vi "FT10xx系列_ITTR_sample_1.0.3.vi"() -> ()   [LabVIEW 2017]
uses:
  National Instruments/LabVIEW 2017/user.lib/smncsftmt/smncsftmt.lvlib
panel:
  in  "模式选择":enum32{"单选选项1", "单选选项2"}(radio)
  out "已连接？":bool
  in  "路径":path=path "D:/Siminics"
  out "error out":errorcluster caption="错误输出"
  in  "统计周期（us）":i32=1000
  in  "采集时间（s）":sgl=1.0
  # "FT10XX系列ITTR"
  # "时间停止："
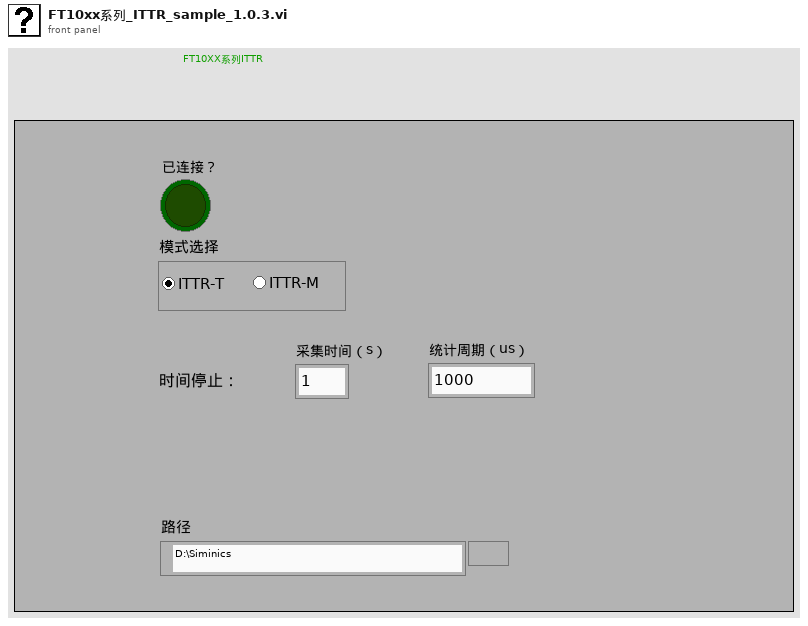
[diagram p1: front panel]
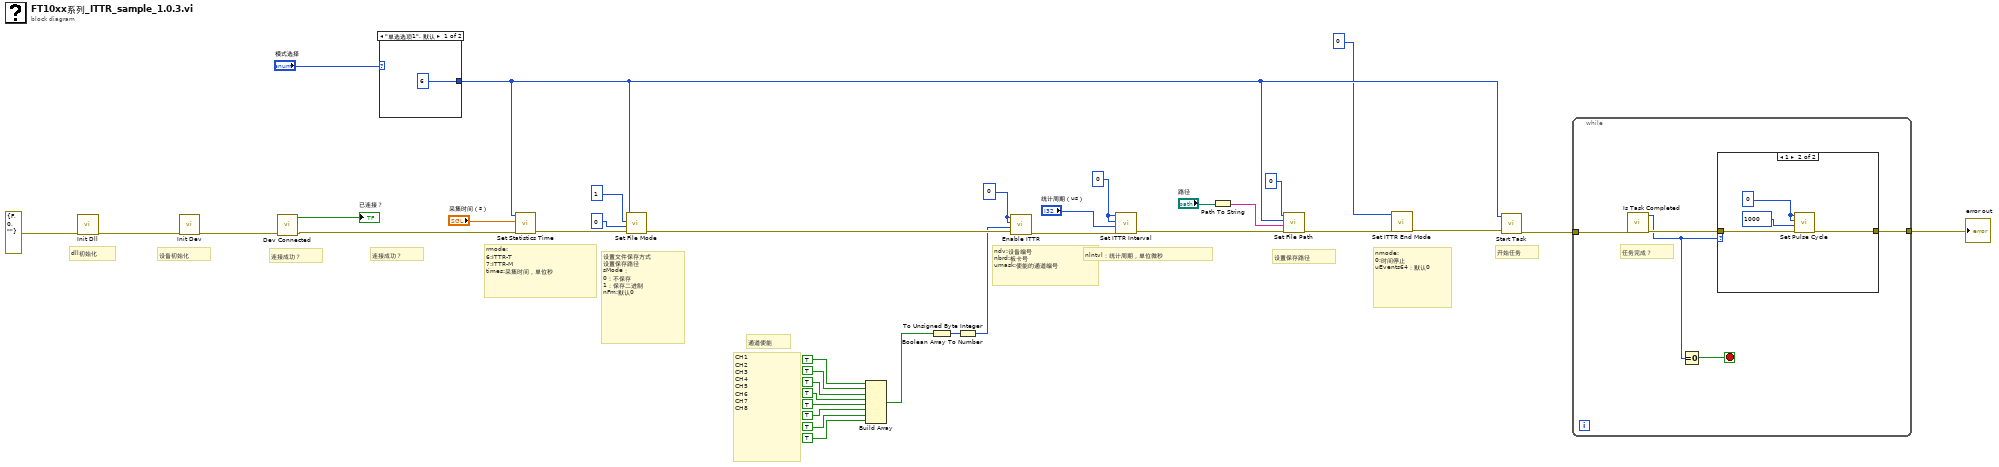
[diagram p0: block diagram]
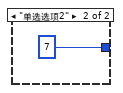
[diagram p2: hidden frame]
diagram:
  w23 = 0
  w24 = 0
  # "通道使能"
  # "CH1\nCH2\nCH3\nCH4\nCH5\nCH6\nCH7\nCH8"
  # "连接成功？"
  # "设备初始化"
  # "dll初始化"
  # "开始任务"
  # "连接成功？"
  # "nmode:\n0:时间停止\nuEvents64：默认0"
  # "设置保存路径"
  # "nlntvl：统计周期，单位微秒"
  # "ndv:设备编号\nnbrd:板卡号\numask:使能的通道编号"
  # "设置文件保存方式\n设置保存路径\nsMode：\n0：不保存\n1：保存二进制\nnFm:默认0"
  # "rmode:\n6:ITTR-T\n7:ITTR-M\ntimes:采集时间，单位秒"
  n1 = call "Init Dll.vi"("error in (no error)"=errorcluster {"status"=FALSE, "code"=0, "source"=""}) -> ("error out"=w18:errorcluster)  [unwired: 9 in, 1 out]
  n2 = call "Init Dev.vi"("error in (no error)"=w18) -> ("error out"=w17:errorcluster)  [unwired: 9 in, 1 out]
  n3 = call "Dev Connected.vi"("error in (no error)"=w17) -> ("error out"=w16:errorcluster, "function return"=→"已连接？":bool)  [unwired: 9 in]
  n4 = case shown="\"单选选项1\", 默认" "模式选择" {
    tunnel: [6 7] -> w20
    frame "单选选项1", Default {
    }
    frame "单选选项2" {
    }
  }
  n5 = call "Set Statistics Time.vi"("error in (no error)"=w16, "Times"="采集时间（s）", "nRunMode"=w20) -> ("error out"=w35:errorcluster)  [unwired: 7 in, 1 out]
  n6 = call "Set File Mode.vi"("error in (no error)"=w35, "nFilterMode"=0, "nSaveMode"=1, "nRunMode"=w20) -> ("error out"=w19:errorcluster)  [unwired: 6 in, 1 out]
  n7 = Build Array(TRUE, TRUE, TRUE, TRUE, TRUE, TRUE, TRUE, TRUE) -> (w4:bool[])
  n8 = Boolean Array To Number(Boolean array=w4) -> (number=w13:u32)
  n9 = To Unsigned Byte Integer(number=w13) -> (unsigned 8bit integer=w3:u8)
  n10 = call "Enable ITTR.vi"("error in (no error)"=w19, "uMask16"=w3, "nBoard"=w24, "nDevId"=w24) -> ("error out"=w34:errorcluster)  [unwired: 6 in, 1 out]
  n11 = call "Set ITTR Interval.vi"("error in (no error)"=w34, "nIntvl"="统计周期（us）", "nBoard"=w23, "nDevId"=w23) -> ("error out"=w32:errorcluster)  [unwired: 6 in, 1 out]
  n12 = Path To String(path="路径") -> (string=w29:string)
  n13 = call "Set File Path.vi"("error in (no error)"=w32, "strFilePath"=w29, "nRunMode"=w20, "nDevId"=0) -> ("error out"=w31:errorcluster)  [unwired: 6 in, 1 out]
  n14 = call "Set ITTR End Mode.vi"("error in (no error)"=w31, "nMode"=0) -> ("error out"=w28:errorcluster)  [unwired: 8 in, 1 out]
  n15 = call "Start Task.vi"("error in (no error)"=w28, "nRunMode"=w20) -> ("error out"=w27:errorcluster)  [unwired: 8 in, 1 out]
  n16 = while {
    tunnel: w27 -> [w43]
    tunnel: [w42] -> w26
    stop <- w39 stop-if-true
    # "任务完成？"
    n17 = call "Is Task Completed.vi"("error in (no error)"=w43) -> ("error out"=w41:errorcluster, "function return"=w40:i32)  [unwired: 9 in]
    n18 = Equal To 0?(x=w40) -> (x = 0?=w39:bool)
    n19 = case shown="1" w40 {
      tunnel: [w44 w47] -> w42
      tunnel: w41 -> [w44 w48]
      frame 0, Default {
      }
      frame 1 {
        w46 = 0
        n20 = call "Set Pulse Cycle.vi"("error in (no error)"=w48, "nCycle"=1000 ("cycle"), "nBoard"=w46, "nDevId"=w46) -> ("error out"=w47:errorcluster)  [unwired: 6 in, 1 out]
      }
    }
  }
  "error out" <- w26
